vi "Migrate - Read v1 Entries.vi"(8 "error in (no error)":errorcluster, 11 "Data Folder":path) -> (0 "error out":errorcluster, 1 "Task Names":string[](array[string]), 2 "Entry IDs":string[](array[string]), 3 "Month File Names":string[](array[string]), 4 "Project Names":string[](array[string]), 5 "Descriptions":string[](array[string]), 6 "Start Times":dbl[](array[numeric]), 7 "End Times":dbl[](array[numeric]))   [LabVIEW 2024]
doc: "Reads every version-1 month file (YYYY-MM.ini) of the data folder. Each section is an entry GUID with keys Task, Project (names), Start Time and End Time (LabVIEW seconds written as numbers - a comma decimal separator is accepted too) and Description. A missing or 0 End Time means the entry is running. Month File Names lists the files that were read, so the caller can remove them once they are migrated. Other .ini files are ignored.\n\nGenerated by: Claude"
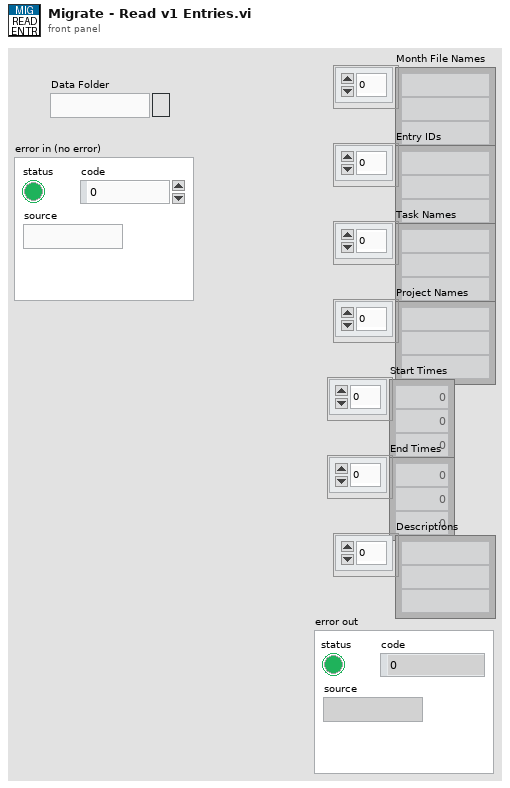
[diagram p1: front panel]
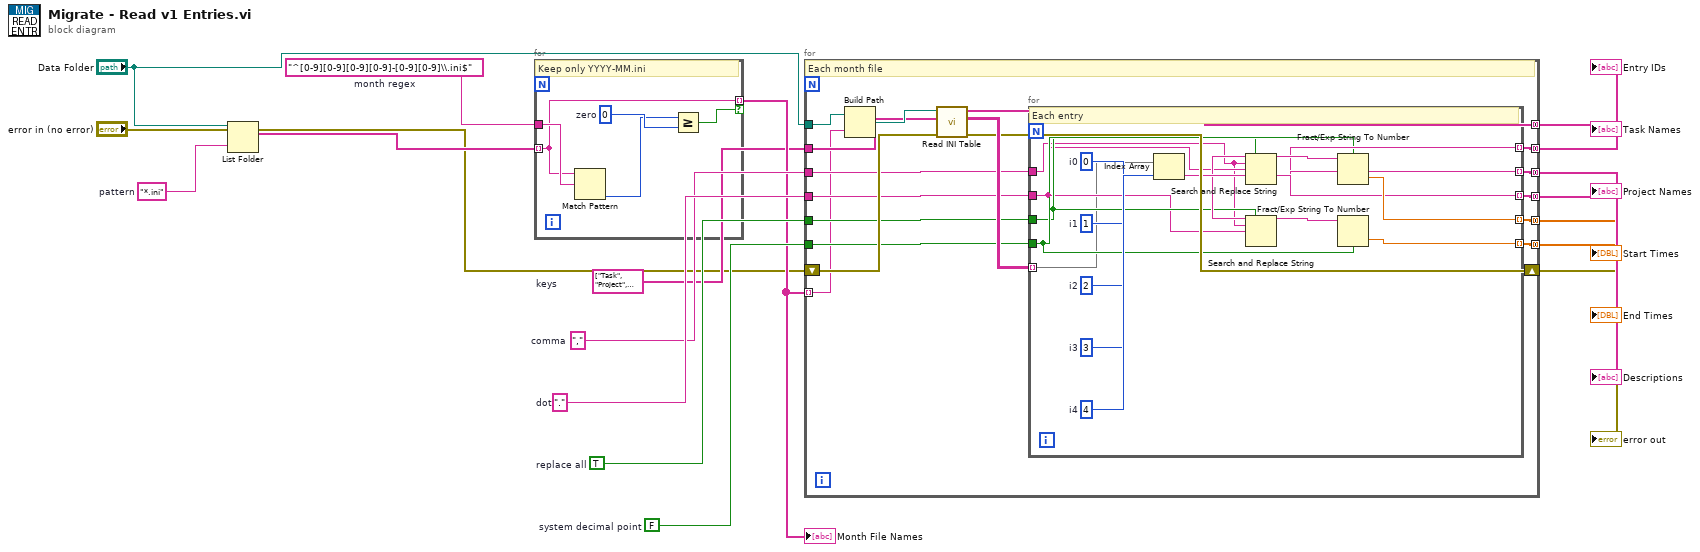
[diagram p0: block diagram]
diagram:
  w11 = FALSE  # system decimal point
  w10 = TRUE  # replace all
  w9 = "."  # dot
  w8 = ","  # comma
  w6 = string[] ["Task", "Project", "Start Time", "End Time", "Description"]  # keys
  w5 = "^[0-9][0-9][0-9][0-9]-[0-9][0-9]\\.ini$"  # month regex
  w3 = "*.ini"  # pattern
  n1 = List Folder(path="Data Folder", pattern=w3) -> (filenames=w4:string[])  [unwired: 2 in, 3 out]
  n2 = for {
    tunnel: w5 -> [w20]
    tunnel: w4 -> [w19] mode=indexing
    tunnel: [w19] -> w7 mode=indexing if=w23
    w22 = 0  # zero
    # "Keep only YYYY-MM.ini"
    n3 = Match Pattern(string=w19, regular expression=w20) -> (offset past match=w21:i32)  [unwired: 1 in, 3 out]
    n4 = Greater Or Equal?(x=w21, y=w22) -> (x >= y?=w23:bool)
  }
  "Month File Names" <- w7
  n5 = for {
    tunnel: "Data Folder" -> [w25]
    tunnel: w6 -> [w26]
    tunnel: w8 -> [w27]
    tunnel: w9 -> [w28]
    tunnel: w10 -> [w29]
    tunnel: w11 -> [w30]
    shift-right: [w32] -> w12
    shift-left: "error in (no error)" -> [w31]
    tunnel: w7 -> [w24] mode=indexing
    tunnel: [w34] -> w13 mode=concatenating
    tunnel: [w36] -> w14 mode=concatenating
    tunnel: [w37] -> w15 mode=concatenating
    tunnel: [w40] -> w18 mode=concatenating
    tunnel: [w38] -> w16 mode=concatenating
    tunnel: [w39] -> w17 mode=concatenating
    # "Each month file"
    n6 = Build Path(base path=w25, name or relative path=w24) -> (appended path=w33:path)
    n7 = call "Read INI Table.vi"("error in (no error)"=w31, "Keys"=w26, "File Path"=w33) -> ("error out"=w32:errorcluster, "Values"=w35:string[][], "Section Names"=w34:string[])  [unwired: 6 in]
    n8 = for {
      tunnel: w27 -> [w42]
      tunnel: w28 -> [w43]
      tunnel: w29 -> [w44]
      tunnel: w30 -> [w45]
      tunnel: w35 -> [w41] mode=indexing
      tunnel: [w51] -> w36 mode=indexing
      tunnel: [w52] -> w37 mode=indexing
      tunnel: [w55] -> w40 mode=indexing
      tunnel: [w58] -> w38 mode=indexing
      tunnel: [w59] -> w39 mode=indexing
      w50 = 4  # i4
      w49 = 3  # i3
      w48 = 2  # i2
      w47 = 1  # i1
      w46 = 0  # i0
      # "Each entry"
      n9 = Index Array(array=w41, index #1=w46, index #2=w47, index #3=w48, index #4=w49, index #5=w50) -> (element #1=w51:string, element #2=w52:string, element #3=w53:string, element #4=w54:string, element #5=w55:string)
      n10 = Search and Replace String(replace all?=w44, input string=w53, search string=w42, replace string=w43) -> (result string=w56:string)  [unwired: 4 in, 3 out]
      n11 = Search and Replace String(replace all?=w44, input string=w54, search string=w42, replace string=w43) -> (result string=w57:string)  [unwired: 4 in, 3 out]
      n12 = Fract/Exp String To Number(use system decimal point (T)=w45, string=w56) -> (number=w58:dbl)  [unwired: 2 in, 1 out]
      n13 = Fract/Exp String To Number(use system decimal point (T)=w45, string=w57) -> (number=w59:dbl)  [unwired: 2 in, 1 out]
    }
  }
  "Entry IDs" <- w13
  "Task Names" <- w14
  "Project Names" <- w15
  "Start Times" <- w16
  "End Times" <- w17
  "Descriptions" <- w18
  "error out" <- w12
